vi "App.Save.vi"(8 "error in (no error)":errorcluster, 10 "selected path":path, 11 "State Variables":T1={"Aliases.All"=[], "Aliases.Outputs"=[], "UI.Sequence#ofColumns"=0, "SysDef.Path"=path "", "UI.SequenceRef"=refnum, "UI.StepInformationRef"=refnum, "UI.AbortRef"=refnum, "UI.GraphRef"=refnum, "UI.ViewRef"=refnum, "UI.IterationsRef"=refnum, "UI.IterationInformationRef"=refnum, "INI.Settings"={"Build Location"=path "C:/Simple Sequence Editor/SequenceRepo", "LoggingLocation"=path ""}, "NIVS.Workspace Event"=refnum, "UI.SkipChannel"=refnum, "NIVS.Launched?"=FALSE, "UI.DurationChannel"=refnum}) -> (0 "error out":errorcluster)   [LabVIEW 2015, in "Simple Sequence Tools - Editor.lvlib"]
uses:
  Simple Sequence Tools - Editor.lvlib
  Types/Main.StateVariables.ctl
  Shared/Types/Channel.Properties.ctl
  Shared/Types/INI.Settings.ctl
  Shared/Types/Saved.Sequence.ctl
  Shared/SubVIs/Main.Constants.vi
  Shared/Simple Sequence Tools - Shared.lvlib
  <vilib>/NI/GXML/GXML.lvlib
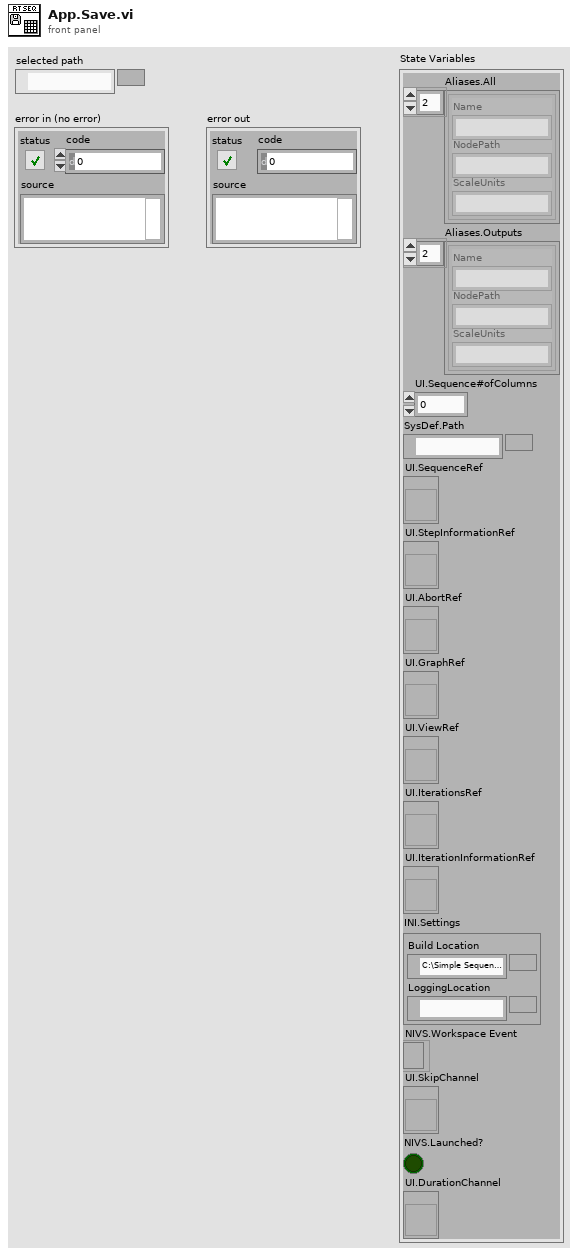
[diagram p1: front panel]
types:
  T1 = typedef "Simple Sequence Tools - Editor.lvlib/Main.StateVariables.ctl" = cluster{"Aliases.All":T2[], "Aliases.Outputs":T2[], "UI.Sequence#ofColumns":i32, "SysDef.Path":path, "UI.SequenceRef":refnum<vi>, "UI.StepInformationRef":refnum<vi>, "UI.AbortRef":refnum<vi>, "UI.GraphRef":refnum<vi>, "UI.ViewRef":refnum<vi>, "UI.IterationsRef":refnum<vi>, "UI.IterationInformationRef":refnum<vi>, "INI.Settings":T3, "NIVS.Workspace Event":refnum<event-registration>, "UI.SkipChannel":refnum<vi>, "NIVS.Launched?":bool, "UI.DurationChannel":refnum<vi>}
  T2 = typedef "Simple Sequence Tools - Shared.lvlib/Channel.Properties.ctl" = cluster{"Name":string, "NodePath":string, "ScaleUnits":string}
  T3 = typedef "Simple Sequence Tools - Shared.lvlib/INI.Settings.ctl" = cluster{"Build Location":path, "LoggingLocation":path}
  T4 = typedef "Simple Sequence Tools - Shared.lvlib/Saved.Sequence.ctl" = cluster{"Output Channels":T2[], "Item Names":string[][], "Step":T2, "Abort":T2, "Iterations":u32, "Iteration":T2, "Skip":T2, "Duration":T2}
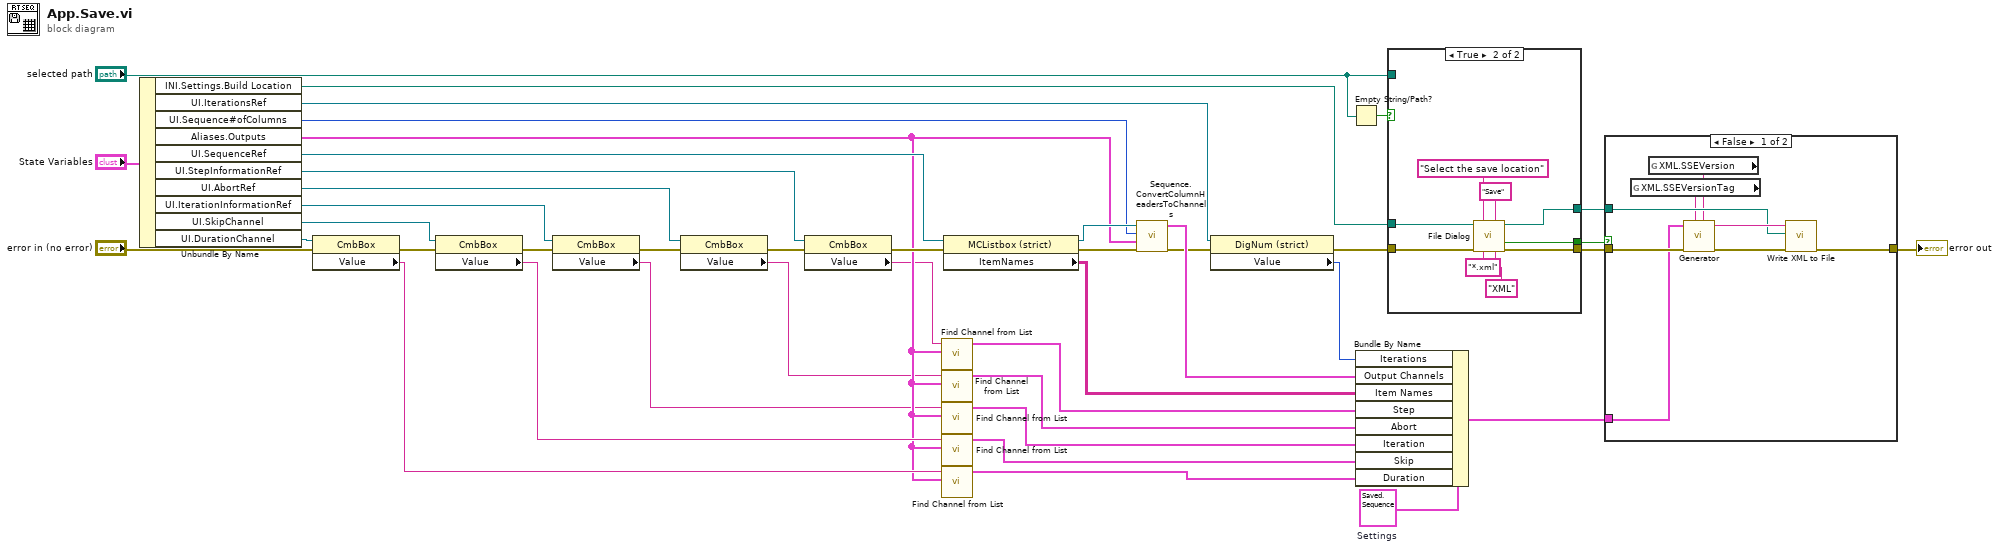
[diagram p0: block diagram]
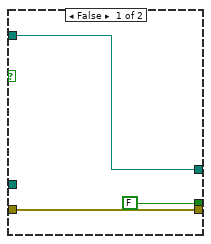
[diagram p2: hidden frame]
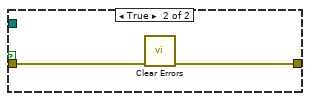
[diagram p3: hidden frame]
diagram:
  w40 = T4 {"Output Channels"=[], "Item Names"=[], "Step"={"Name"="", "NodePath"="", "ScaleUnits"=""}, "Abort"={"Name"="", "NodePath"="", "ScaleUnits"=""}, "Iterations"=0, "Iteration"={"Name"="", "NodePath"="", "ScaleUnits"=""}, "Skip"={"Name"="", "NodePath"="", "ScaleUnits"=""}, "Duration"={"Name"="", "NodePath"="", "ScaleUnits"=""}}  # Settings
  n1 = Unbundle By Name("State Variables") -> ("INI.Settings.Build Location"=w17:path, "UI.IterationsRef"=w29:refnum<vi>, "UI.Sequence#ofColumns"=w22:i32, "Aliases.Outputs"=w7:T2[], "UI.SequenceRef"=w30:refnum<vi>, "UI.StepInformationRef"=w36:refnum<vi>, "UI.AbortRef"=w37:refnum<vi>, "UI.IterationInformationRef"=w28:refnum<vi>, "UI.SkipChannel"=w16:refnum<vi>, "UI.DurationChannel"=w12:refnum<vi>)
  n2 = property class="CmbBox"(reference=w12, error in="error in (no error)") -> (error out=w13:errorcluster, "Value"=w11:string)  [unwired: 1 out]
  n3 = property class="CmbBox"(reference=w16, error in=w13) -> (error out=w15:errorcluster, "Value"=w9:string)  [unwired: 1 out]
  n4 = property class="CmbBox"(reference=w28, error in=w15) -> (error out=w27:errorcluster, "Value"=w6:string)  [unwired: 1 out]
  n5 = property class="CmbBox"(reference=w37, error in=w27) -> (error out=w38:errorcluster, "Value"=w4:string)  [unwired: 1 out]
  n6 = property class="CmbBox"(reference=w36, error in=w38) -> (error out=w39:errorcluster, "Value"=w2:string)  [unwired: 1 out]
  n7 = call "Find Channel from List.vi"("Aliases.Outputs"=w7, "Value"=w2) -> ("Channel"=w1:T2)  [unwired: 9 in]
  n8 = call "Find Channel from List.vi"("Aliases.Outputs"=w7, "Value"=w4) -> ("Channel"=w3:T2)  [unwired: 9 in]
  n9 = call "Find Channel from List.vi"("Aliases.Outputs"=w7, "Value"=w6) -> ("Channel"=w5:T2)  [unwired: 9 in]
  n10 = call "Find Channel from List.vi"("Aliases.Outputs"=w7, "Value"=w9) -> ("Channel"=w8:T2)  [unwired: 9 in]
  n11 = call "Find Channel from List.vi"("Aliases.Outputs"=w7, "Value"=w11) -> ("Channel"=w10:T2)  [unwired: 9 in]
  n12 = property class="MCListbox (strict)"(reference=w30, error in=w39) -> (reference out=w23:refnum<vi>, error out=w26:errorcluster, "ItemNames"=w20:string[][])
  n13 = call "Sequence.ConvertColumnHeadersToChannels.vi"("error in (no error)"=w26, "Aliases.Outputs"=w7, "UI.Sequence#ofColumns"=w22, "UI.SequenceRef"=w23) -> ("error out"=w25:errorcluster, "Output Channels"=w41:T2[])  [unwired: 5 in, 1 out]
  n14 = property class="DigNum (strict)"(reference=w29, error in=w25) -> (error out=w24:errorcluster, "Value"=w21:u32)  [unwired: 1 out]
  n15 = Empty String/Path?(string/path="selected path") -> (empty?=w19:bool)
  n16 = Bundle By Name(cluster=w40, "Iterations"=w21, "Output Channels"=w41, "Item Names"=w20, "Step"=w1, "Abort"=w3, "Iteration"=w5, "Skip"=w8, "Duration"=w10) -> (w42:T4)
  n17 = case shown="True" w19 {
    tunnel: [FALSE ("cancelled") w53] -> w34
    tunnel: [w43 w52] -> w33
    tunnel: [w45 w48] -> w32
    tunnel: w24 -> [w45 w46]
    tunnel: "selected path" -> [w43 _]
    tunnel: w17 -> [_ w47]
    frame False {
    }
    frame True {
      n18 = call "File Dialog"("start path"=w47, "prompt"="Select the save location", "button label"="Save", "error in"=w46, "pattern (all files)"="*.xml", "pattern label"="XML") -> ("selected path"=w52:path, "cancelled"=w53:bool, "error out"=w48:errorcluster)  [unwired: 6 in, 1 out]
    }
  }
  n19 = case shown="False" w34 {
    tunnel: [w58 w63] -> w31
    tunnel: w32 -> [w62 w64]
    tunnel: w33 -> [w59 _]
    tunnel: w42 -> [w57 _]
    frame False {
      n20 = global read "Main.Constants.vi" "XML.SSEVersionTag"() -> (w56:string)
      n21 = global read "Main.Constants.vi" "XML.SSEVersion"() -> (w55:string)
      n22 = call <vilib>:"Generator.vi"("Version String"=w55, "Version Tag Name"=w56, "error in"=w62, "Variant"=w57) -> ("error out"=w60:errorcluster, "XML String Out"=w61:string)  [unwired: 6 in]
      n23 = call <vilib>:"Write XML to File.vi"("error in"=w60, "XML File Path"=w59, "XML Input"=w61) -> ("error out"=w58:errorcluster)  [unwired: 8 in]
    }
    frame True {
      n24 = call <vilib>:"Clear Errors.vi"("error in (no error)"=w64) -> ("error out"=w63:errorcluster)  [unwired: 5 in, 1 out]
    }
  }
  "error out" <- w31
